vi "MQTT Data - Decode String.vi"(7 "Encoded String":u8[](array[numeric]), 9 "From UTF8?":bool=TRUE, 11 "error in (no error)":errorcluster) -> (4 "remaining data":u8[](array[numeric]), 8 "String":string, 15 "error out":errorcluster)   [LabVIEW 2019, in "KoRE-MQTT.lvlib"]
doc: "Copyright (c) 2025 KoRElibs.com\nSPDX-License-Identifier: EUPL-1.2\n\nThis VI is licensed under the European Union Public License (EUPL) Version 1.2. You may use this VI unmodified in proprietary works. If you distribute a modified version of this file, the modified file must be released under the EUPL-1.2. Full license: https://joinup.ec.europa.eu/asset/eupl/eupl/1.2/"
uses:
  KoRE-MQTT.lvlib
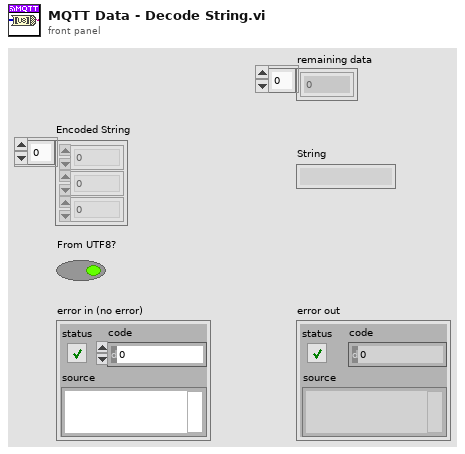
[diagram p1: front panel]
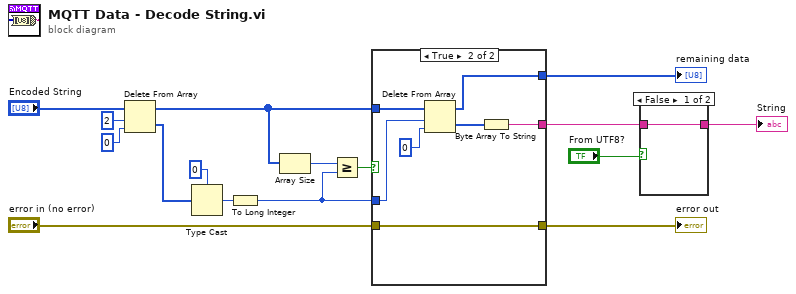
[diagram p0: block diagram]
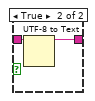
[diagram p2: hidden frame]
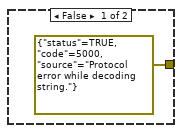
[diagram p3: hidden frame]
diagram:
  n1 = Delete From Array(array="Encoded String", length=2, index=0) -> (deleted portion=w13:u8[], array with subset deleted=w9:u8[])
  n2 = Type Cast(type=u16 0, x=w13) -> (*(type *) &x=w11:u16)
  n3 = To Long Integer(number=w11) -> (32bit integer=w4:i32)
  n4 = Array Size(array=w9) -> (size(s)=w5:i32)
  n5 = Greater Or Equal?(x=w5, y=w4) -> (x >= y?=w8:bool)
  n6 = case shown="True" w8 {
    tunnel: [_ w24] -> w3
    tunnel: [_ w21] -> w10
    tunnel: w9 -> [_ w20]
    tunnel: "error in (no error)" -> [_ w19]
    tunnel: [errorcluster {"status"=TRUE, "code"=5000, "source"="Protocol error while decoding string."} ("error in (no error)") w19] -> w6
    tunnel: w4 -> [_ w18]
    frame False {
    }
    frame True {
      n7 = Delete From Array(array=w20, length=w18, index=0) -> (deleted portion=w22:u8[], array with subset deleted=w21:u8[])
      n8 = Byte Array To String(unsigned byte array=w22) -> (string=w24:string)
    }
  }
  "error out" <- w6
  "remaining data" <- w10
  n9 = case shown="False" "From UTF8?" {
    tunnel: w3 -> [w25 w27]
    tunnel: [w25 w26] -> w2
    frame False {
    }
    frame True {
      n10 = UTF-8 to Text(11:w27) -> (3:w26:string)  [unwired: 2 in, 1 out]
    }
  }
  "String" <- w2
